vi "Run Test (Array Path).vi"(4 "timeout (2000 ms)":i32=2000, 5 "Test Report":refnum<class "Test Report.lvclass">, 6 "Verbose":bool, 7 "Report Path":path, 8 "error in":errorcluster, 9 "Inspect Recursively (T)":bool=TRUE, 10 "Paths":path[](array[path]), 11 "Interactive (T)":bool=TRUE) -> (0 "error out":errorcluster, 3 "Test Results":refnum<class "Test Result.lvclass">)   [LabVIEW 2020, in "Caraya.lvlib"]
doc: "\"Run Tests\" from a Array of Path (folders or VIs):\n- Dynamically discovers Caraya unit tests and runs them based on array of VI paths or folders\n- Outputs results in a UI ans/or Test Report (J-Unit or text)\n\n(Not compatible with RT targets or RunTime Engine)"
uses:
  Caraya.lvlib
  classes/Test Report/Test Report.lvclass
  classes/Test Result/Test Result.lvclass
  classes/Test Runner.Folder/Test Runner.Folder.lvclass
  C:/projects/caraya/src/classes/Test Runner/Test Runner.lvclass
  <userlib>/_OpenG.lib/file/file.llb/Valid Path - Array__ogtk.vi
  <userlib>/_OpenG.lib/file/file.llb/File Exists - Array__ogtk.vi
  classes/Test Runner/Test Runner.lvclass
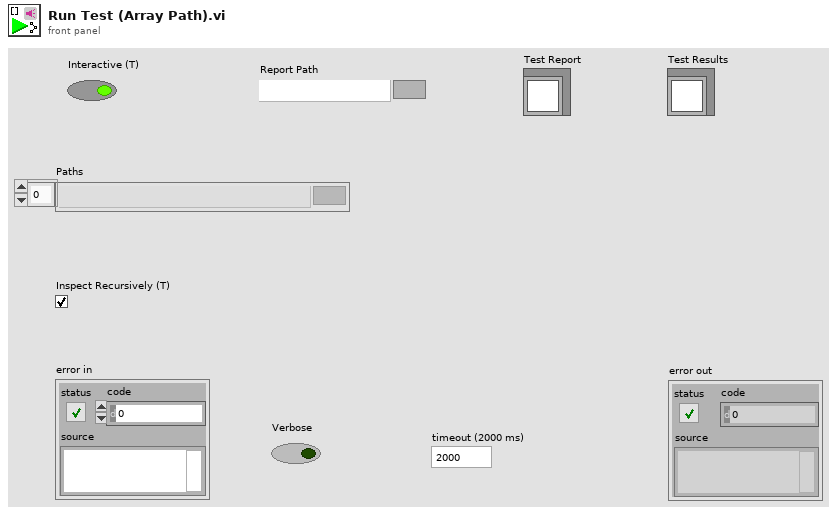
[diagram p1: front panel]
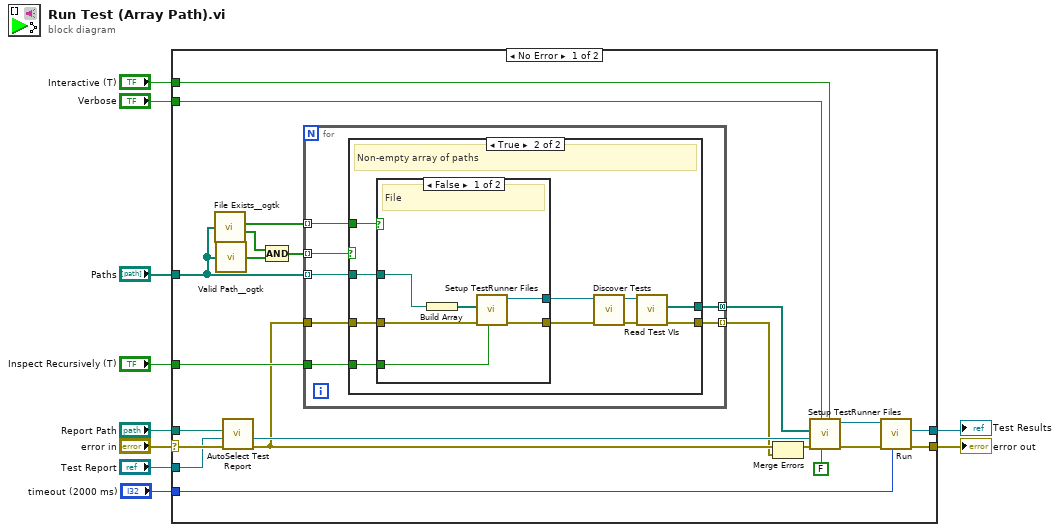
[diagram p0: block diagram]
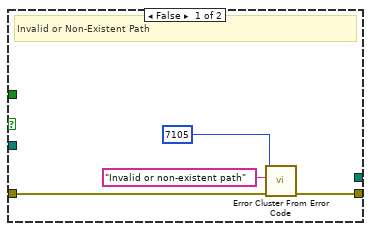
[diagram p2: hidden frame]
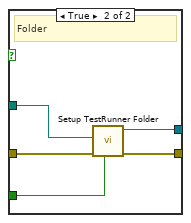
[diagram p3: hidden frame]
diagram:
  n1 = case shown="No Error" "error in" {
    selector: "error in" -> [w32 w65]
    tunnel: [w20 w65] -> w10
    tunnel: "Verbose" -> [w16 _]
    tunnel: "Interactive (T)" -> [w17 _]
    tunnel: "Test Report" -> [w30 _]
    tunnel: "Paths" -> [w28 _]
    tunnel: "Report Path" -> [w31 _]
    tunnel: "Inspect Recursively (T)" -> [w18 _]
    tunnel: "timeout (2000 ms)" -> [w12 _]
    tunnel: [w11 _] -> w1
    frame No Error {
      n2 = call-poly <userlib>:"File Exists__ogtk.vi"("file paths"=w28) -> ("is directory"=w25:bool[], "exists"=w29:bool[])  [unwired: 6 in]
      n3 = call-poly <userlib>:"Valid Path__ogtk.vi"("array of paths"=w28) -> ("valid"=w27:bool[])
      n4 = call "AutoSelect Test Report.vi"("error in (no error)"=w32, "Test Report in"=w30, "Report Path"=w31) -> ("error out"=w14:errorcluster, "Test Report out"=w19:refnum<class "Test Report.lvclass">)  [unwired: 7 in]
      n5 = Compound Arithmetic op=AND(w29, w27) -> (w26:bool[])
      n6 = for {
        tunnel: [w39] -> w13 mode=indexing
        tunnel: w14 -> [w38]
        tunnel: w18 -> [w37]
        tunnel: w28 -> [w36] mode=indexing
        tunnel: w26 -> [w35] mode=indexing
        tunnel: w25 -> [w34] mode=indexing
        tunnel: [w33] -> w24 mode=concatenating
        n7 = case shown="True" w35 {
          tunnel: [w42 w45] -> w39
          tunnel: w38 -> [w43 w53]
          tunnel: w37 -> [_ w52]
          tunnel: w36 -> [_ w51]
          tunnel: w34 -> [_ w50]
          tunnel: [_ w44] -> w33
          frame False {
            # "Invalid or Non-Existent Path"
            n8 = call <vilib>:"Error Cluster From Error Code.vi"("error in (no error)"=w43, "error message (\"\")"="Invalid or non-existent path" ("error message (\"\")"), "error code (0)"=7105 ("code")) -> ("error out"=w42:errorcluster)  [unwired: 6 in]
          }
          frame True {
            # "Non-empty array of paths"
            n9 = case shown="False" w50 {
              tunnel: [w58 w60] -> w47
              tunnel: [w57 w61] -> w48
              tunnel: w53 -> [w59 w64]
              tunnel: w51 -> [w56 w62]
              tunnel: w52 -> [w55 w63]
              frame False {
                # "File"
                n10 = Build Array(w56) -> (w54:path[])
                n11 = call "Setup TestRunner Files.vi"("Inspect Recursively (T)"=w55, "error in (no error)"=w59, "Paths"=w54) -> ("error out"=w58:errorcluster, "Test Runner.Folder out"=w57:refnum<class "Test Runner.Folder.lvclass">)  [unwired: 7 in]
              }
              frame True {
                # "Folder"
                n12 = call "Setup TestRunner Folder.vi"("Inspect Recursively (T)"=w63, "error in (no error)"=w64, "Directory to search"=w62) -> ("error out"=w60:errorcluster, "Test Runner.Folder out"=w61:refnum<class "Test Runner.Folder.lvclass">)  [unwired: 7 in]
              }
            }
            n13 = call "Discover Tests.vi"("error in (no error)"=w47, "Test Runner in"=w48) -> ("error out"=w46:errorcluster, "Test Runner out"=w49:refnum<class "Test Runner.Folder.lvclass">)  [unwired: 8 in]
            n14 = call "Read Test VIs.vi"("error in (no error)"=w46, "Test Runner in"=w49) -> ("error out"=w45:errorcluster, "Test VIs"=w44:path[])  [unwired: 7 in, 1 out]
          }
        }
      }
      n15 = Merge Errors(w14, w13) -> (w23:errorcluster)
      n16 = call "Setup TestRunner Files.vi"("Interactive (T)"=w17, "Inspect Recursively (T)"=FALSE, "Verbose (F)"=w16, "error in (no error)"=w23, "Test Report"=w19, "Paths"=w24) -> ("error out"=w21:errorcluster, "Test Runner.Folder out"=w22:refnum<class "Test Runner.Folder.lvclass">)  [unwired: 4 in]
      n17 = call "Run.vi"("timeout"=w12, "error in (no error)"=w21, "Test Runner in"=w22) -> ("error out"=w20:errorcluster, "Test Suite Results"=w11:refnum<class "Test Result.lvclass">)  [unwired: 6 in, 1 out]
    }
    frame Error {
    }
  }
  "error out" <- w10
  "Test Results" <- w1
